vi "midiin_main.vi"() -> ()   [LabVIEW 2020]
uses:
  shared/midi message type.ctl
  shared/midi note number.ctl
  midi-callback-userevent/midi-callback-userevent.lvclass/midi-callback-userevent.ctl
  midi/midi.lvclass
  midi-callback-userevent/midi-callback-userevent.lvclass
  midi-ui/midi-ui.lvclass
panel:
  out "Keyboard Picture":picture
  out "Note Value":T1
  out "Message Type":T2
  out "delta time (ms)":u32
  out "data 1":i32
  out "Data2":i32
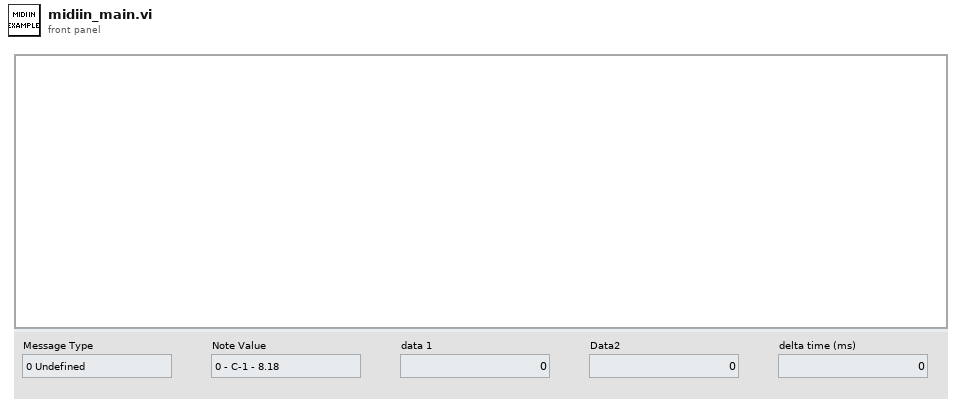
[diagram p1: front panel]
types:
  T1 = typedef "midi note number.ctl" = enum8{"0 - C-1 - 8.18", "1 - C#-1 - 8.66", "2 - D-1 - 9.18", "3 - D#-1 - 9.72", "4 - E-1 - 10.30", "5 - F-1 - 10.91", "6 - F#-1 - 11.56", "7 - G-1 - 12.25", "8 - G#-1 - 12.98", "9 - A-1 - 13.75", "10 - A#-1 - 14.57", "11 - B-1 - 15.43", "12 - C0 - 16.35", "13 - C#0 - 17.32", "14 - D0 - 18.35", "15 - D#0 - 19.45", "16 - E0 - 20.60", "17 - F0 - 21.83", "18 - F#0 - 23.12", "19 - G0 - 24.50", "20 - G#0 - 25.96", "21 - A0 - 27.50", "22 - A#0 - 29.14", "23 - B0 - 30.87", "24 - C1 - 32.70", "25 - C#1 - 34.65", "26 - D1 - 36.71", "27 - D#1 - 38.89", "28 - E1 - 41.20", "29 - F1 - 43.65", "30 - F#1 - 46.25", "31 - G1 - 49.00", "32 - G#1 - 51.91", "33 - A1 - 55.00", "34 - A#1 - 58.27", "35 - B1 - 61.74", "36 - C2 - 65.41", "37 - C#2 - 69.30", "38 - D2 - 73.42", "39 - D#2 - 77.78", "40 - E2 - 82.41", "41 - F2 - 87.31", "42 - F#2 - 92.50", "43 - G2 - 98.00", "44 - G#2 - 103.83", "45 - A2 - 110.00", "46 - A#2 - 116.54", "47 - B2 - 123.47", "48 - C3 - 130.81", "49 - C#3 - 138.59", "50 - D3 - 146.83", "51 - D#3 - 155.56", "52 - E3 - 164.81", "53 - F3 - 174.61", "54 - F#3 - 185.00", "55 - G3 - 196.00", "56 - G#3 - 207.65", "57 - A3 - 220.00", "58 - A#3 - 233.08", "59 - B3 - 246.94", "60 - C4 - 261.63", "61 - C#4 - 277.18", "62 - D4 - 293.66", "63 - D#4 - 311.13", "64 - E4 - 329.63", "65 - F4 - 349.23", "66 - F#4 - 369.99", "67 - G4 - 392.00", "68 - G#4 - 415.30", "69 - A4 - 440.00", "70 - A#4 - 466.16", "71 - B4 - 493.88", "72 - C5 - 523.25", "73 - C#5 - 554.37", "74 - D5 - 587.33", "75 - D#5 - 622.25", "76 - E5 - 659.25", "77 - F5 - 698.46", "78 - F#5 - 739.99", "79 - G5 - 783.99", "80 - G#5 - 830.61", "81 - A5 - 880.00", "82 - A#5 - 932.33", "83 - B5 - 987.77", "84 - C6 - 1046.50", "85 - C#6 - 1108.73", "86 - D6 - 1174.66", "87 - D#6 - 1244.51", "88 - E6 - 1318.51", "89 - F6 - 1396.91", "90 - F#6 - 1479.98", "91 - G6 - 1567.98", "92 - G#6 - 1661.22", "93 - A6 - 1760.00", "94 - A#6 - 1864.66", "95 - B6 - 1975.53", "96 - C7 - 2093.00", "97 - C#7 - 2217.46", "98 - D7 - 2349.32", "99 - D#7 - 2489.02", "100 - E7 - 2637.02", "101 - F7 - 2793.83", "102 - F#7 - 2959.96", "103 - G7 - 3135.96", "104 - G#7 - 3322.44", "105 - A7 - 3520.00", "106 - A#7 - 3729.31", "107 - B7 - 3951.07", "108 - C8 - 4186.01", "109 - C#8 - 4434.92", "110 - D8 - 4698.63", "111 - D#8 - 4978.03", "112 - E8 - 5274.04", "113 - F8 - 5587.65", "114 - F#8 - 5919.91", "115 - G8 - 6271.93", "116 - G#8 - 6644.88", "117 - A8 - 7040.00", "118 - A#8 - 7458.62", "119 - B8 - 7902.13", "120 - C9 - 8372.02", "121 - C#9 - 8869.84", "122 - D9 - 9397.27", "123 - D#9 - 9956.06", "124 - E9 - 10548.08", "125 - F9 - 11175.30", "126 - F#9 - 11839.82", "127 - G9 - 12543.85"}
  T2 = typedef "midi message type.ctl" = enum8{"0 Undefined", "1 Undefined", "2 Undefined", "3 Undefined", "4 Undefined", "5 Undefined", "6 Undefined", "7 Undefined", "Note Off", "Note On", "Polyphonic Key Pressure", "Control Change", "Program Change", "Channel Pressure", "Pitch Bend", "System Message"}
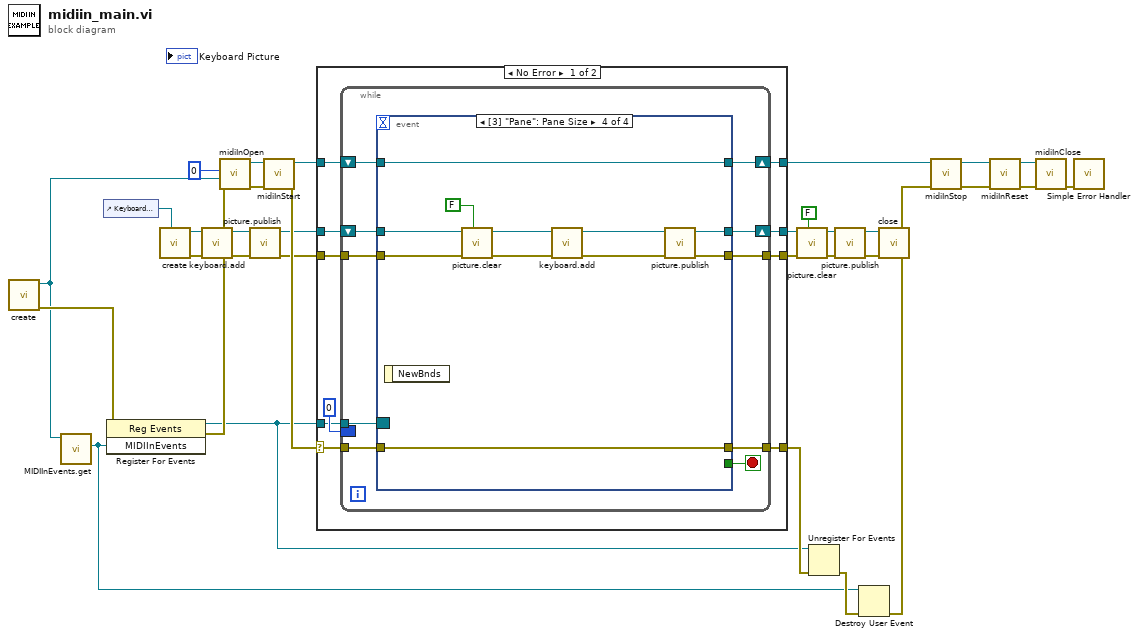
[diagram p0: block diagram]
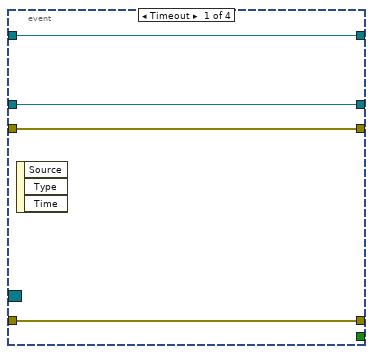
[diagram p2: hidden frame]
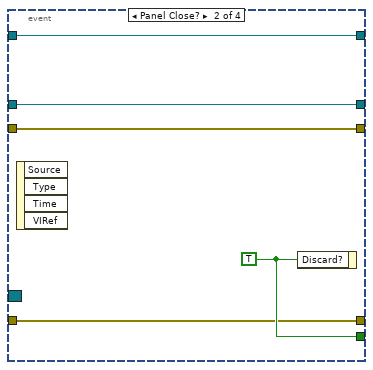
[diagram p3: hidden frame]
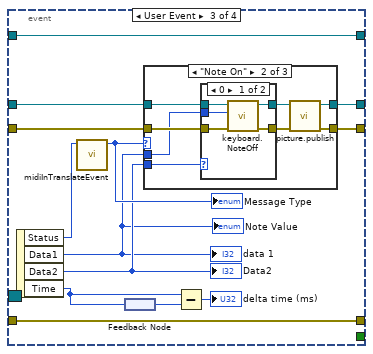
[diagram p4: hidden frame]
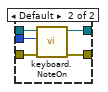
[diagram p6: hidden frame]
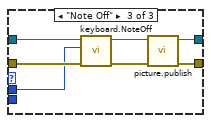
[diagram p7: hidden frame]
diagram:
  n1 = call "create.vi"() -> ("error out"=w20:errorcluster, "midi-callback-userevent out"=w18:refnum<class "midi-callback-userevent.lvclass">)  [unwired: 10 in]
  n2 = call "MIDIInEvents.get.vi"("midi-callback-userevent"=w18) -> ("MIDIInEvents"=w17:refnum<user-event>)  [unwired: 10 in]
  n3 = control-ref of="Keyboard Picture"() -> (w13:refnum<vi>)
  n4 = register-events(error in=w20, w17) -> (reference out=w16:refnum<event-registration>, error out=w19:errorcluster)  [unwired: 1 in]
  n5 = call "create.vi"("Picture Control"=w13) -> ("error out"=w14:errorcluster, "midi-ui out"=w15:refnum<class "midi-ui.lvclass">)  [unwired: 9 in]
  n6 = call "keyboard.add.vi"("error in (no error)"=w14, "midi-ui in"=w15) -> ("error out"=w4:errorcluster, "midi-ui out"=w3:refnum<class "midi-ui.lvclass">)  [unwired: 8 in]
  n7 = call "midiInOpen.vi"("error in"=w19, "midi-callback-userevent"=w18, "MIDI Device ID"=u32 0) -> ("error out"=w21:errorcluster, "midi out"=w22:refnum<class "midi.lvclass">)  [unwired: 7 in]
  n8 = call "picture.publish.vi"("error in"=w4, "midi-ui in"=w3) -> ("error out"=w2:errorcluster, "midi-ui out"=w1:refnum<class "midi-ui.lvclass">)  [unwired: 8 in]
  n9 = call "midiInStart.vi"("error in"=w21, "midi in"=w22) -> ("error out"=w29:errorcluster, "midi out"=w30:refnum<class "midi.lvclass">)  [unwired: 8 in]
  n10 = case shown="No Error" w29 {
    selector: w29 -> [w41 w117]
    tunnel: w30 -> [w43 w116]
    tunnel: [w42 w117] -> w32
    tunnel: [w40 w116] -> w28
    tunnel: w16 -> [w38 _]
    tunnel: w2 -> [w37 w114]
    tunnel: w1 -> [w36 w115]
    tunnel: [w35 w115] -> w10
    tunnel: [w34 w114] -> w9
    frame No Error {
      n11 = while {
        shift-right: [w53] -> w40
        shift-left: w43 -> [w52]
        tunnel: w41 -> [w51]
        tunnel: [w50] -> w42
        border: u32 0 ("Time") -> [_]
        tunnel: w38 -> [w48]
        tunnel: w37 -> [w47]
        shift-right: [w45] -> w35
        shift-left: w36 -> [w46]
        tunnel: [w44] -> w34
        stop <- w49 stop-if-true
        n12 = event shown="[3] \"Pane\": Pane Size" {
          selector: w48 -> [_ _ _ _]
          dyn-events: _ -> [_ _ _ _]
          timeout: _ -> [_ _ _ _]
          tunnel: [w57 w62 w75 w113] -> w53
          tunnel: w52 -> [w57 w62 w75 w113]
          tunnel: w51 -> [w56 w60 w74 w107]
          tunnel: [w56 w60 w74 w107] -> w50
          tunnel: [_ w61 _ _] -> w49
          tunnel: w47 -> [w54 w58 w67 w111]
          tunnel: w46 -> [w55 w59 w70 w112]
          tunnel: [w55 w59 w69 w103] -> w45
          tunnel: [w54 w58 w68 w104] -> w44
          event Timeout {
            n13 = event-data() -> ()  [unwired: 1 in, 3 out]
          }
          event Panel Close? {
            w61 = TRUE ("Discard?")
            n14 = event-data() -> ()  [unwired: 1 in, 4 out]
            n15 = event-data("Discard?"=w61) -> ()  [unwired: 1 in, 1 out]
          }
          event User Event {
            n16 = event-data() -> ("Status"=w66:i32, "Data1"=w63:i32, "Data2"=w64:i32, "Time"=w72:u32)  [unwired: 1 in]
            "Data2" <- w64
            "data 1" <- w63
            "Note Value" <- w63
            n17 = call "midiInTranslateEvent.vi"("status"=w66) -> ("Message Type"=w65:T2)  [unwired: 9 in, 1 out]
            "Message Type" <- w65
            n18 = feedback-in #1(w72) -> ()
            n19 = feedback #1() -> (w73:u32)
            n20 = case shown="\"Note On\"" w65 {
              tunnel: w70 -> [w77 w80 w100]
              tunnel: [w77 w84 w102] -> w69
              tunnel: [w76 w85 w101] -> w68
              tunnel: w67 -> [w76 w81 w97]
              tunnel: w63 -> [_ w79 w96]
              tunnel: w64 -> [_ w78 _]
              frame Default {
              }
              frame "Note On" {
                n21 = case shown="0" w78 {
                  tunnel: [w88 w95] -> w83
                  tunnel: [w89 w94] -> w82
                  tunnel: w81 -> [w87 w93]
                  tunnel: w80 -> [w90 w92]
                  tunnel: w79 -> [w86 w91]
                  frame 0 {
                    n22 = call "keyboard.NoteOff.vi"("error in (no error)"=w87, "Note"=w86, "midi-ui in"=w90) -> ("error out"=w89:errorcluster, "midi-ui out"=w88:refnum<class "midi-ui.lvclass">)  [unwired: 7 in]
                  }
                  frame Default {
                    n23 = call "keyboard.NoteOn.vi"("error in (no error)"=w93, "Note"=w91, "midi-ui in"=w92) -> ("error out"=w94:errorcluster, "midi-ui out"=w95:refnum<class "midi-ui.lvclass">)  [unwired: 7 in]
                  }
                }
                n24 = call "picture.publish.vi"("error in"=w82, "midi-ui in"=w83) -> ("error out"=w85:errorcluster, "midi-ui out"=w84:refnum<class "midi-ui.lvclass">)  [unwired: 8 in]
              }
              frame "Note Off" {
                n25 = call "keyboard.NoteOff.vi"("error in (no error)"=w97, "Note"=w96, "midi-ui in"=w100) -> ("error out"=w98:errorcluster, "midi-ui out"=w99:refnum<class "midi-ui.lvclass">)  [unwired: 7 in]
                n26 = call "picture.publish.vi"("error in"=w98, "midi-ui in"=w99) -> ("error out"=w101:errorcluster, "midi-ui out"=w102:refnum<class "midi-ui.lvclass">)  [unwired: 8 in]
              }
            }
            n27 = Subtract(x=w72, y=w73) -> (x-y=→"delta time (ms)":u32)
          }
          event Pane Size {
            n28 = event-data() -> ()  [unwired: 1 in, 1 out]
            n29 = call "picture.clear.vi"("Keep Keyboard? (T)"=FALSE, "error in"=w111, "midi-ui in"=w112) -> ("error out"=w108:errorcluster, "midi-ui out"=w109:refnum<class "midi-ui.lvclass">)  [unwired: 7 in]
            n30 = call "keyboard.add.vi"("error in (no error)"=w108, "midi-ui in"=w109) -> ("error out"=w105:errorcluster, "midi-ui out"=w106:refnum<class "midi-ui.lvclass">)  [unwired: 8 in]
            n31 = call "picture.publish.vi"("error in"=w105, "midi-ui in"=w106) -> ("error out"=w104:errorcluster, "midi-ui out"=w103:refnum<class "midi-ui.lvclass">)  [unwired: 8 in]
          }
        }
      }
    }
    frame Error {
    }
  }
  n32 = call "picture.clear.vi"("Keep Keyboard? (T)"=FALSE, "error in"=w9, "midi-ui in"=w10) -> ("error out"=w7:errorcluster, "midi-ui out"=w8:refnum<class "midi-ui.lvclass">)  [unwired: 7 in]
  n33 = Unregister For Events(event registration refnum=w16, error in=w32) -> (error out=w33:errorcluster)
  n34 = call "picture.publish.vi"("error in"=w7, "midi-ui in"=w8) -> ("error out"=w6:errorcluster, "midi-ui out"=w5:refnum<class "midi-ui.lvclass">)  [unwired: 8 in]
  n35 = Destroy User Event(user event=w17, error in=w33) -> (error out=w27:errorcluster)
  n36 = call "close.vi"("error in (no error)"=w6, "midi-ui in"=w5) -> ()  [unwired: 9 in, 1 out]
  n37 = call "midiInStop.vi"("error in"=w27, "midi in"=w28) -> ("error out"=w26:errorcluster, "midi out"=w25:refnum<class "midi.lvclass">)  [unwired: 8 in]
  n38 = call "midiInReset.vi"("error in"=w26, "midi in"=w25) -> ("error out"=w24:errorcluster, "midi out"=w23:refnum<class "midi.lvclass">)  [unwired: 8 in]
  n39 = call "midiInClose.vi"("error in"=w24, "midi in"=w23) -> ("error out"=w31:errorcluster)  [unwired: 8 in, 1 out]
  n40 = call <vilib>:"Simple Error Handler.vi"("error in (no error)"=w31) -> ()  [unwired: 4 in, 5 out]
